vi "Check status.vi"(8 "error in":errorcluster, 11 "VISA resource name":refnum<visa-resource-name>) -> (0 "error out":errorcluster, 1 "RESULT":bool, 2 "Current":string, 3 "Voltage":string)   [LabVIEW 2021]
uses:
  HI-POT_Driver/GPT-9800_GSB_L8.5/GPT-9000.lvlib
panel:
  out "Return  the test status":string
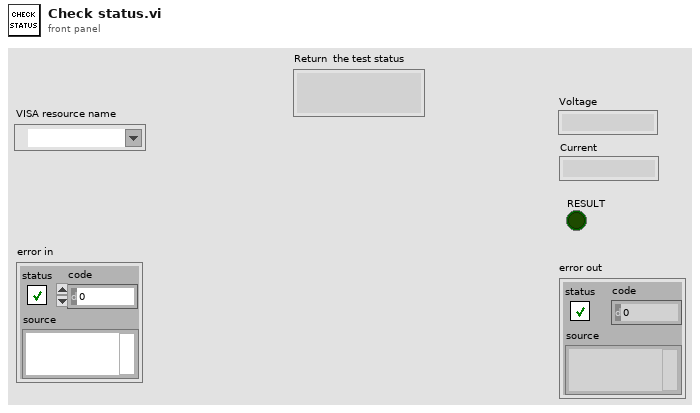
[diagram p1: front panel]
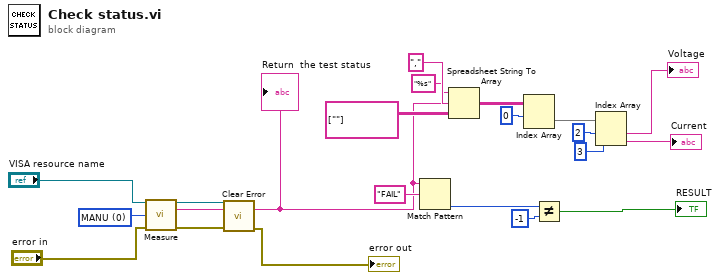
[diagram p0: block diagram]
diagram:
  w10 = u8 0 items=["MANU", "AUTO"] ("Function Mode Numeric")
  n1 = call "Measure.vi"("VISA resource name"="VISA resource name", "Function Mode Numeric"=w10, "error in"="error in") -> ("VISA resource name out"=w3:refnum<visa-resource-name>, "Return  the test status"=w8:string, "error out"=w2:errorcluster)  [unwired: 9 in, 1 out]
  "Return  the test status" <- w8
  n2 = call "Clear Error.vi"("error in (no error)"=w2, "VISA resource name"=w3) -> ("error out"=→"error out":errorcluster)  [unwired: 8 in, 1 out]
  n3 = Match Pattern(string=w8, regular expression="FAIL") -> (offset past match=w12:i32)  [unwired: 1 in, 3 out]
  n4 = Spreadsheet String To Array(delimiter (Tab)=",", format string="%s", spreadsheet string=w8, array type (2D Dbl)=string[][] [[""]]) -> (array=w18:string[][])
  n5 = Index Array(array=w18, index (row)=0) -> (element=w16:string[])  [unwired: 1 in]
  n6 = Not Equal?(x=w12, y=-1) -> (x != y?=→"RESULT":bool)
  n7 = Index Array(array=w16, index #1=2 ("index"), index #2=3 ("index")) -> (element #1=→"Voltage":string, element #2=→"Current":string)
